vi "SeqEditor_getConPanekids_Clust30.vi"(11 "Array":T1(array[cluster])) -> (3 "Array 2":T1(array[cluster]))   [LabVIEW 2017, in "NLTest.lvclass"]
uses:
  NLTest.lvclass
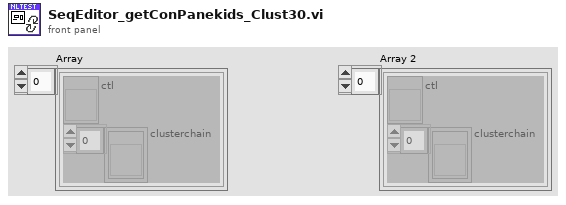
[diagram p1: front panel]
types:
  T1 = cluster{"ctl":refnum<vi>, "clusterchain":refnum<vi>[]}[]
  T2 = cluster{"ctl":refnum<vi>, "clusterchain":refnum<vi>[]}
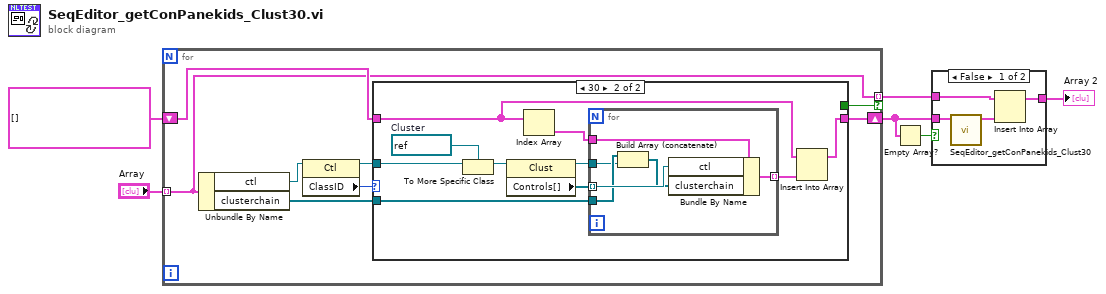
[diagram p0: block diagram]
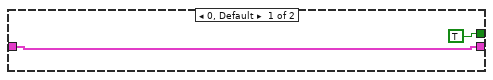
[diagram p3: hidden frame]
diagram:
  n1 = for {
    tunnel: "Array" -> [w7] mode=indexing
    tunnel: [w7] -> w3 mode=indexing if=w13
    shift-right: [w10] -> w2
    shift-left: T1 [] ("Array 3") -> [w11]
    n2 = Unbundle By Name(w7) -> ("ctl"=w9:refnum<vi>, "clusterchain"=w8:refnum<vi>[])
    n3 = property class="Ctl"(reference=w9) -> (reference out=w12:refnum<vi>, "ClassID"=w14:u32)  [unwired: 1 in, 1 out]
    n4 = case shown="30" w14 {
      tunnel: [TRUE _] -> w13
      tunnel: w12 -> [_ w25]
      tunnel: w11 -> [w15 w19]
      tunnel: [w15 w23] -> w10
      tunnel: w8 -> [_ w21]
      frame 0, Default {
      }
      frame 30 {
        w26 = refnum<vi> refnum  # Cluster
        n5 = To More Specific Class(target class=w26, reference=w25) -> (specific class reference=w24:refnum<vi>)  [unwired: 1 in, 1 out]
        n6 = property class="Clust"(reference=w24) -> (reference out=w20:refnum<vi>, "Controls[]"=w22:refnum<vi>[])  [unwired: 1 in, 1 out]
        n7 = Index Array(array=w19) -> (element=w18:T2)  [unwired: 1 in]
        n8 = for {
          tunnel: w22 -> [w32] mode=indexing
          tunnel: w21 -> [w31]
          tunnel: w20 -> [w30]
          tunnel: w18 -> [w28]
          tunnel: [w27] -> w17 mode=indexing
          n9 = Build Array (concatenate)(w31, w30) -> (w29:refnum<vi>[])
          n10 = Bundle By Name(cluster=w28, "ctl"=w32, "clusterchain"=w29) -> (w27:T2)
        }
        n11 = Insert Into Array(array=w19, new element=w17) -> (w23:T1)  [unwired: 1 in]
      }
    }
  }
  n12 = Empty Array?(array=w2) -> (empty?=w5:bool)
  n13 = case shown="False" w5 {
    tunnel: [w34 w37] -> w4
    tunnel: w3 -> [w36 w37]
    tunnel: w2 -> [w35 _]
    frame False {
      n14 = call "SeqEditor_getConPanekids_Clust30.vi"("Array"=w35) -> ("Array 2"=w33:T1)  [unwired: 10 in]
      n15 = Insert Into Array(array=w36, new element=w33) -> (w34:T1)  [unwired: 1 in]
    }
    frame True {
    }
  }
  "Array 2" <- w4
